vi "CE Unflatten value.vi"(5 "Flattened DBL?":bool, 6 "error in":errorcluster, 7 "type":T1=enum."DBL Number", 8 "flattened data":string, 9 "dbl":dbl format="%.2f") -> (0 "error out":errorcluster, 3 "values out":T2={"type"=enum."DBL Number", "dbl"=0.0, "cdb"=0.0+0.0i, "str"="", "1d dbl"=[], "1d cdb"=[], "1d str"=[], "2d dbl"=[], "2d cdb"=[], "2d str"=[]} {"2d cdb" format="%.2f"; "2d dbl" format="%.2f"; "1d cdb" format="%.2f"; "1d dbl" format="%.2f"; "cdb" format="%.2f"; "dbl" format="%.2f"})   [LabVIEW 2021]
doc: "::: CalcExpress Toolkit :::\nCopyright (c) 2000-2026 Konstantin Shifershteyn. All rights reserved."
uses:
  vi.lib/addons/CalcExpress/cetypes.llb/CalcExpress Data Type.ctl
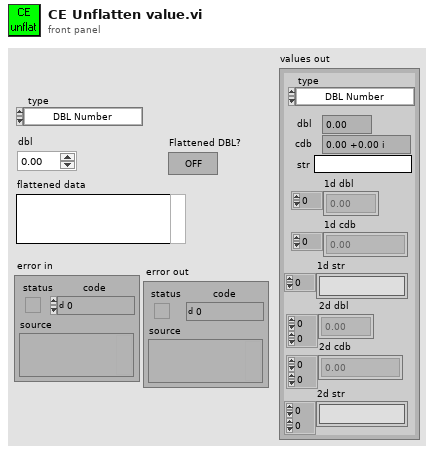
[diagram p1: front panel]
types:
  T1 = typedef "CalcExpress Data Type.ctl" = enum32{"String", "DBL Number", "identifier", "1D Array of DBL", "2D Array of DBL", "CDB Number", "1D Array of CDB", "2D Array of CDB", "1D Array of String", "2D Array of String", "Unknown data type"}
  T2 = cluster{"type":T1, "dbl":dbl, "cdb":cdb, "str":string, "1d dbl":dbl[], "1d cdb":cdb[], "1d str":string[], "2d dbl":dbl[][], "2d cdb":cdb[][], "2d str":string[][]}
  T3 = cluster{"type":enum32{"String", "DBL Number", "identifier", "1D Array of DBL", "2D Array of DBL", "CDB Number", "1D Array of CDB", "2D Array of CDB", "1D Array of String", "2D Array of String", "Unknown data type"}, "dbl":dbl, "cdb":cdb, "str":string, "1d dbl":dbl[], "1d cdb":cdb[], "1d str":string[], "2d dbl":dbl[][], "2d cdb":cdb[][], "2d str":string[][]}
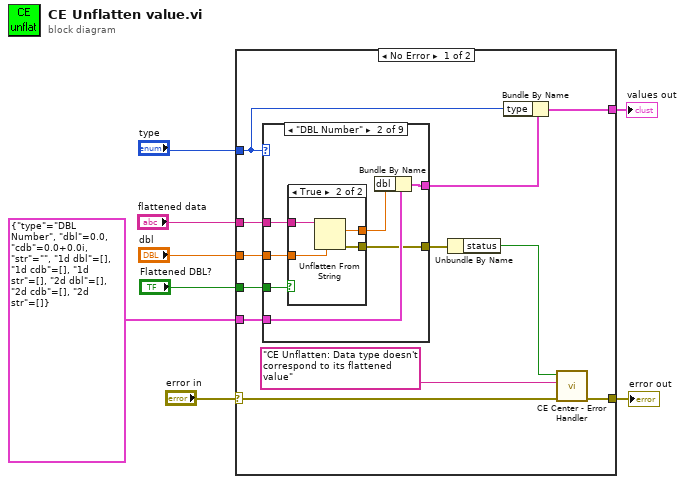
[diagram p0: block diagram]
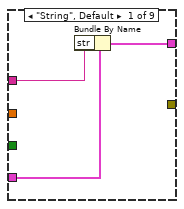
[diagram p2: hidden frame]
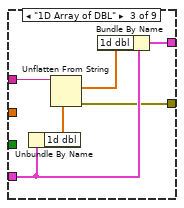
[diagram p4: hidden frame]
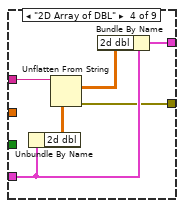
[diagram p5: hidden frame]
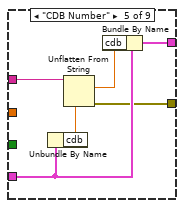
[diagram p6: hidden frame]
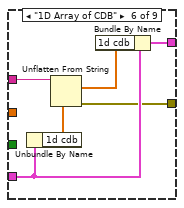
[diagram p7: hidden frame]
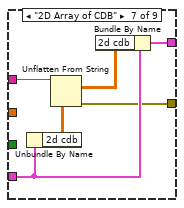
[diagram p8: hidden frame]
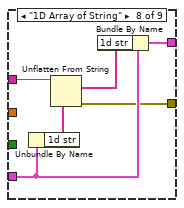
[diagram p9: hidden frame]
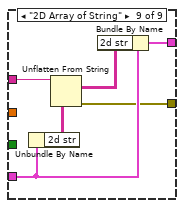
[diagram p10: hidden frame]
diagram:
  n1 = case shown="No Error" "error in" {
    selector: "error in" -> [w11 w78]
    tunnel: "flattened data" -> [w20 _]
    tunnel: T3 {"type"=enum."DBL Number", "dbl"=0.0, "cdb"=0.0+0.0i, "str"="", "1d dbl"=[], "1d cdb"=[], "1d str"=[], "2d dbl"=[], "2d cdb"=[], "2d str"=[]} ("values in") -> [w19 w79]
    tunnel: "type" -> [w17 _]
    tunnel: [w16 w79] -> w5
    tunnel: [w15 w78] -> w4
    tunnel: "Flattened DBL?" -> [w13 _]
    tunnel: "dbl" -> [w12 _]
    frame No Error {
      n2 = case shown="\"DBL Number\"" w17 {
        tunnel: w20 -> [w23 w28 w39 w45 w51 w57 w63 w69 w75]
        tunnel: w19 -> [w22 w29 w37 w43 w49 w55 w61 w67 w73]
        tunnel: [w21 w30 w41 w47 w53 w59 w65 w71 w77] -> w18
        tunnel: w13 -> [_ w26 _ _ _ _ _ _ _]
        tunnel: w12 -> [_ w25 _ _ _ _ _ _ _]
        tunnel: [_ w24 w36 w42 w48 w54 w60 w66 w72] -> w10
        frame "String", Default {
          n3 = Bundle By Name(cluster=w22, "str"=w23) -> (w21:T3)
        }
        frame "DBL Number" {
          n4 = case shown="True" w26 {
            tunnel: w28 -> [_ w35]
            tunnel: [w31 w34] -> w27
            tunnel: w25 -> [w31 w32]
            tunnel: [_ w33] -> w24
            frame False {
            }
            frame True {
              n5 = Unflatten From String(type=w32, binary string=w35) -> (value=w34:dbl, error out=w33:errorcluster)  [unwired: 3 in, 1 out]
            }
          }
          n6 = Bundle By Name(cluster=w29, "dbl"=w27) -> (w30:T3)
        }
        frame "1D Array of DBL" {
          n7 = Unbundle By Name(w37) -> ("1d dbl"=w38:dbl[])
          n8 = Unflatten From String(type=w38, binary string=w39) -> (value=w40:dbl[], error out=w36:errorcluster)  [unwired: 3 in, 1 out]
          n9 = Bundle By Name(cluster=w37, "1d dbl"=w40) -> (w41:T3)
        }
        frame "2D Array of DBL" {
          n10 = Unbundle By Name(w43) -> ("2d dbl"=w44:dbl[][])
          n11 = Unflatten From String(type=w44, binary string=w45) -> (value=w46:dbl[][], error out=w42:errorcluster)  [unwired: 3 in, 1 out]
          n12 = Bundle By Name(cluster=w43, "2d dbl"=w46) -> (w47:T3)
        }
        frame "CDB Number" {
          n13 = Unbundle By Name(w49) -> ("cdb"=w50:cdb)
          n14 = Unflatten From String(type=w50, binary string=w51) -> (value=w52:cdb, error out=w48:errorcluster)  [unwired: 3 in, 1 out]
          n15 = Bundle By Name(cluster=w49, "cdb"=w52) -> (w53:T3)
        }
        frame "1D Array of CDB" {
          n16 = Unbundle By Name(w55) -> ("1d cdb"=w56:cdb[])
          n17 = Unflatten From String(type=w56, binary string=w57) -> (value=w58:cdb[], error out=w54:errorcluster)  [unwired: 3 in, 1 out]
          n18 = Bundle By Name(cluster=w55, "1d cdb"=w58) -> (w59:T3)
        }
        frame "2D Array of CDB" {
          n19 = Unbundle By Name(w61) -> ("2d cdb"=w62:cdb[][])
          n20 = Unflatten From String(type=w62, binary string=w63) -> (value=w64:cdb[][], error out=w60:errorcluster)  [unwired: 3 in, 1 out]
          n21 = Bundle By Name(cluster=w61, "2d cdb"=w64) -> (w65:T3)
        }
        frame "1D Array of String" {
          n22 = Unbundle By Name(w67) -> ("1d str"=w68:string[])
          n23 = Unflatten From String(type=w68, binary string=w69) -> (value=w70:string[], error out=w66:errorcluster)  [unwired: 3 in, 1 out]
          n24 = Bundle By Name(cluster=w67, "1d str"=w70) -> (w71:T3)
        }
        frame "2D Array of String" {
          n25 = Unbundle By Name(w73) -> ("2d str"=w74:string[][])
          n26 = Unflatten From String(type=w74, binary string=w75) -> (value=w76:string[][], error out=w72:errorcluster)  [unwired: 3 in, 1 out]
          n27 = Bundle By Name(cluster=w73, "2d str"=w76) -> (w77:T3)
        }
      }
      n28 = Unbundle By Name(w10) -> ("status"=w9:bool)
      n29 = Bundle By Name(cluster=w18, "type"=w17) -> (w16:T3)
      n30 = call "CE Center - Error Handler.vi"("error before"=w11, "CE message"="CE Unflatten: Data type doesn't correspond to its flattened value", "CE error status"=w9) -> ("error out"=w15:errorcluster)  [unwired: 6 in]
    }
    frame Error {
    }
  }
  "values out" <- w5
  "error out" <- w4
